vi "Initialize TreeBrowserWF.vi"(7 "Generate?":bool, 8 "error in (no error)":errorcluster, 9 "Input Channels":T1[](array[typedef]) {"Data Type" items=["Signed", "Unsigned", "IEEE Float"]}, 10 "Node Pointer":T2, 11 "TreeBrowserRef":refnum<k24>) -> (0 "error out":errorcluster, 2 "Channels":variant, 3 "TreeBrowserRef 2":refnum<k24>)   [LabVIEW 2015, in "Protection and Rolling Counter Addon System Explorer.lvlib"]
uses:
  Protection and Rolling Counter Addon System Explorer.lvlib
  <vilib>/NI Veristand/Custom Device API/Custom Device Pointer.ctl
  NationalInstruments.VeriStand.SystemStorage
  Shared/Types/InputChannelConfiguration.ctl
  NationalInstruments.VeriStand.SystemStorageUI
  NationalInstruments.VeriStand
  <vilib>/NI Veristand/Custom Device API/Custom Device API.lvlib
  Shared/Protection and Rolling Counter Addon Shared.lvlib
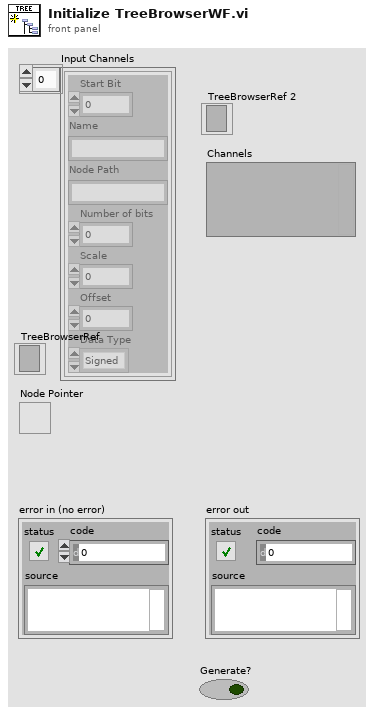
[diagram p1: front panel]
types:
  T1 = typedef "Protection and Rolling Counter Addon Shared.lvlib/InputChannelConfiguration.ctl" = cluster{"Start Bit":i32, "Name":string, "Node Path":string, "Number of bits":i32, "Scale":dbl, "Offset":dbl, "Data Type":u32}
  T2 = typedef "Custom Device API.lvlib/Custom Device Pointer.ctl" = refnum<k24>
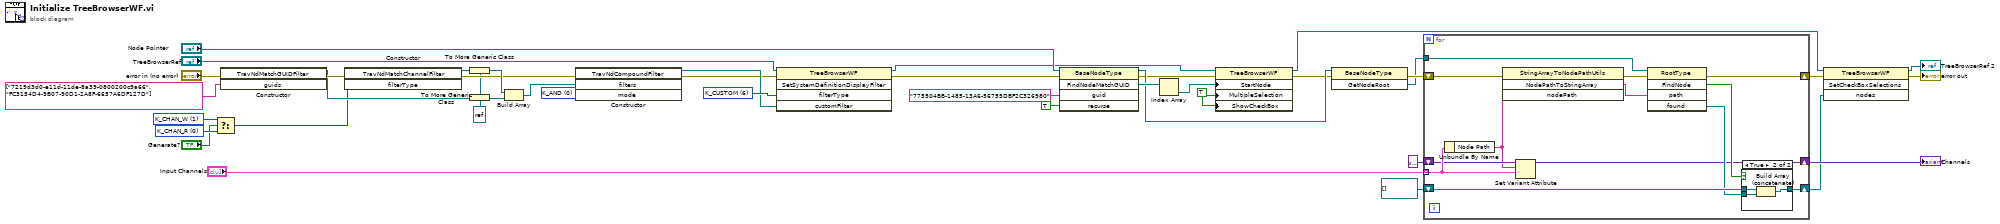
[diagram p0: block diagram]
diagram:
  w16 = refnum<k24> refnum
  w21 = 0 items=["K_AND", "K_OR"] ("mode")
  w24 = u8 0 items=["K_CHAN_R", "K_CHAN_W", "K_CHAN_VOLT", "K_CHAN_FAULT"] ("filterType")
  w25 = u8 1 items=["K_CHAN_R", "K_CHAN_W", "K_CHAN_VOLT", "K_CHAN_FAULT"] ("filterType")
  w36 = TRUE ("MultipleSelection")
  w30 = u8 6 items=["K_CHAN_R", "K_CHAN_W", "K_CHAN_RW", "K_CHAN_VOLT", "K_CHAN_FAULT", "K_ALL", "K_CUSTOM", "K_CHAN_R_VIS", "K_CHAN_W_VIS", "K_CHAN_RW_VIS", "K_CHAN_VOLT_VIS", "K_CHAN_FAULT_VIS", "K_WAVE", "K_WAVE_VIS", "K_WAVE_DBL", "K_WAVE_CDB", "K_WAVE_DBL_VIS", "K_WAVE_CDB_VIS"] ("filterType")
  n1 = Select(t=w25, s="Generate?", f=w24) -> (s? t:f=w11:u8)
  n2 = constructor class="TravNdMatchGUIDFilter"(error in="error in (no error)", "guids"=string[] ["7219d3d0-e11d-11de-8a39-0800200c9a66", "FC3154D4-9B07-90D1-2A8F-6657A6DF127D"]) -> (reference out=w13:refnum<k24>, error out=w14:errorcluster)  [unwired: 2 in, 2 out]
  n3 = constructor class="TravNdMatchChannelFilter"(error in=w14, "filterType"=w11) -> (reference out=w15:refnum<k24>, error out=w17:errorcluster)  [unwired: 2 in, 2 out]
  n4 = To More Generic Class(target class=w16, reference=w15) -> (generic class reference=w19:refnum<k24>)
  n5 = To More Generic Class(target class=w16, reference=w13) -> (generic class reference=w20:refnum<k24>)
  n6 = Build Array(w19, w20) -> (w18:refnum<k24>[])
  n7 = constructor class="TravNdCompoundFilter"(error in=w17, "filters"=w18, "mode"=w21) -> (reference out=w12:refnum<k24>, error out=w9:errorcluster)  [unwired: 2 in, 3 out]
  n8 = invoke class="TreeBrowserWF" method="SetSystemDefinitionDisplayFilter"(reference="TreeBrowserRef", error in=w9, "filterType"=w30, "customFilter"=w12) -> (reference out=w7:refnum<k24>, error out=w4:errorcluster)  [unwired: 1 in, 3 out]
  n9 = invoke class="BaseNodeType" method="FindNodeMatchGUID"(reference="Node Pointer", error in=w4, "guid"="775504BB-1485-13A6-56755DBF2C326980", "recurse"=TRUE) -> (reference out=w5:T2, error out=w3:errorcluster, "FindNodeMatchGUID"=w28:refnum<k24>[])  [unwired: 1 in, 2 out]
  n10 = Index Array(array=w28) -> (element=w27:refnum<k24>)  [unwired: 1 in]
  n11 = property class="TreeBrowserWF"(reference=w7, error in=w3, "StartNode"=w27, "MultipleSelection"=w36, "ShowCheckBox"=w36) -> (reference out=w6:refnum<k24>, error out=w2:errorcluster)
  n12 = invoke class="BaseNodeType" method="GetNodeRoot"(reference=w5, error in=w2) -> (error out=w41:errorcluster, "GetNodeRoot"=w40:refnum<k24>)  [unwired: 1 in, 1 out]
  n13 = for {
    shift-right: [w51] -> w35
    shift-left: w41 -> [w43]
    tunnel: "Input Channels" -> [w46] mode=indexing
    tunnel: w40 -> [w54]
    shift-right: [w48] -> w37
    shift-left: refnum<k24>[] [] -> [w49]
    shift-right: [w44] -> w39
    shift-left: variant -> [w45]
    n14 = Unbundle By Name(w46) -> ("Node Path"=w42:string)
    n15 = invoke class="StringArrayToNodePathUtils" method="NodePathToStringArray"(error in=w43, "nodePath"=w42) -> (error out=w52:errorcluster, "NodePathToStringArray"=w53:string[])  [unwired: 2 in, 2 out]
    n16 = Set Variant Attribute(Variant=w45, name=w42, value=w46) -> (Variant out=w44:variant)  [unwired: 1 in, 2 out]
    n17 = invoke class="RootType" method="FindNode"(reference=w54, error in=w52, "path"=w53) -> (error out=w51:errorcluster, "FindNode"=w50:bool, "found"=w47:refnum<k24>)  [unwired: 2 in, 2 out]
    n18 = case shown="True" w50 {
      tunnel: w49 -> [w55 w58]
      tunnel: [w55 w56] -> w48
      tunnel: w47 -> [_ w57]
      frame False {
      }
      frame True {
        n19 = Build Array (concatenate)(w58, w57) -> (w56:refnum<k24>[])
      }
    }
  }
  "Channels" <- w39
  n20 = invoke class="TreeBrowserWF" method="SetCheckBoxSelections"(reference=w6, error in=w35, "nodes"=w37) -> (reference out=→"TreeBrowserRef 2":refnum<k24>, error out=→"error out":errorcluster)  [unwired: 1 in, 2 out]
